vi "ZM-CP-init.vi"(8 "error in (no error)":errorcluster, 11 "ZM-CP-FL-file_logger in":refnum<class "ZM-CP-FL-file_logger.lvclass">) -> (0 "error out":errorcluster, 3 "ZM-CP-FL-file_logger out":refnum<class "ZM-CP-FL-file_logger.lvclass">)   [LabVIEW 2020, in "ZM-CP-FL-file_logger.lvlib" / "ZM-CP-FL-file_logger.lvclass"]
doc: "Initialises the communication protocol (dynamic dispatch): writes opened = TRUE through the private accessor Write opened. This is the real default of the parent; a child overrides it, calls the parent and then runs its own hook."
uses:
  ZM-CP-FL-file_logger.lvclass
  ZM-CP-communication_protocol/ZM-CP-communication_protocol/ZM-CP-communication_protocol.lvclass
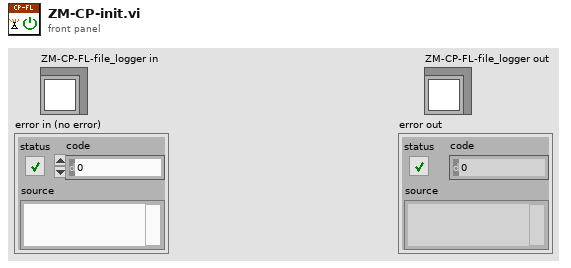
[diagram p1: front panel]
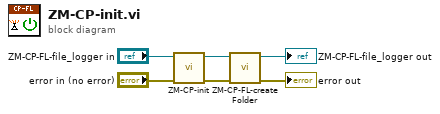
[diagram p0: block diagram]
diagram:
  n1 = call-parent "ZM-CP-init.vi"("error in (no error)"="error in (no error)", "ZM-CP-communication_protocol in"="ZM-CP-FL-file_logger in") -> ("error out"=w1:errorcluster, "ZM-CP-communication_protocol out"=w3:refnum<class "ZM-CP-FL-file_logger.lvclass">)  [unwired: 8 in]
  n2 = call "ZM-CP-FL-createFolder.vi"("error in (no error)"=w1, "ZM-CP-communication_protocol in"=w3) -> ("error out"=→"error out":errorcluster, "ZM-CP-communication_protocol out"=→"ZM-CP-FL-file_logger out":refnum<class "ZM-CP-FL-file_logger.lvclass">)  [unwired: 8 in]
